vi "VIH HelpGen - Build.vi"(8 "error in":errorcluster, 9 "Allowed files":path[](array[path]), 10 "Items Array":T3[](array[typedef]), 11 "Project Tree":T2) -> (0 "error out":errorcluster, 2 "Items out":T1, 3 "dup Project Tree":T2)   [LabVIEW 2014]
doc: "::: VI Helpeks :::\nCopyright (c) 2000-2026 Konstantin Shifershteyn. All rights reserved."
uses:
  _VIH HelpGen - Palette.llb/VIH HelpGen Typedef - Palette - Item Info Cluster.ctl
  _VIH HelpGen - Palette.llb/VIH HelpGen Typedef - Palette - Item Type Enum.ctl
  _VIH Project Manager.llb/VIH Project Tree Typedef - Tree Refnum.ctl
panel:
  # "VI Helpeks\nCopyright (c) 2012-2026 Konstantin Shifershteyn"
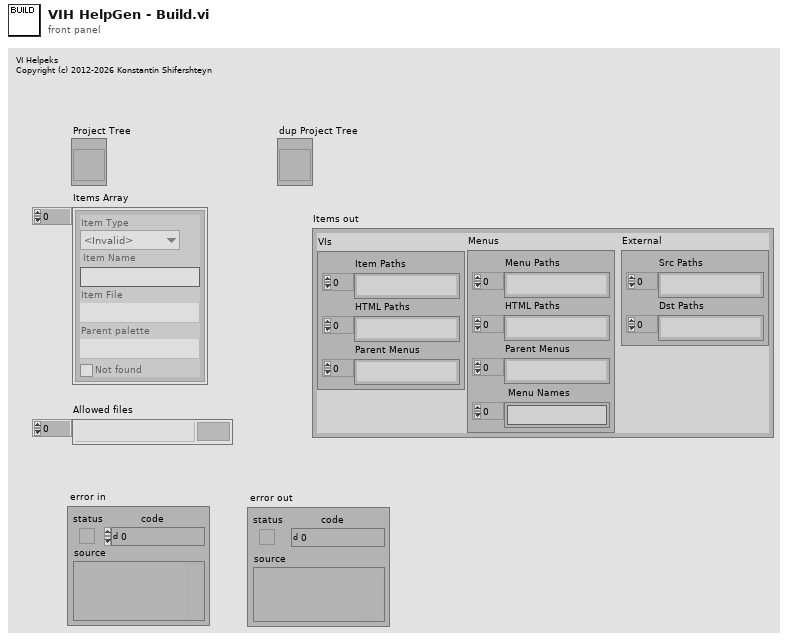
[diagram p1: front panel]
types:
  T1 = cluster{"VIs":cluster{"Item Paths":path[], "HTML Paths":path[], "Parent Menus":path[]}, "Menus":cluster{"Menu Paths":path[], "HTML Paths":path[], "Parent Menus":path[], " Menu Names":string[]}, "External":cluster{"Src Paths":path[], "Dst Paths":path[]}}
  T2 = typedef "VIH Project Tree Typedef - Tree Refnum.ctl" = refnum<vi>
  T3 = typedef "VIH HelpGen Typedef - Palette - Item Info Cluster.ctl" = cluster{"Item Type":T4, "Item Name":string, "Item File":path, "Parent palette":path, "Not found":bool}
  T4 = typedef "VIH HelpGen Typedef - Palette - Item Type Enum.ctl" = enum32{"<Invalid>", "<unknown>", "VI", "Menu", "LV Func", "Express VI", "Poly VI", "CTL", "HTML"}
  T5 = enum16{"nop", "Start", "Stop", "Run-prep", "Run-VI", "Run-Menu"}
  T6 = cluster{"Menu Paths":path[], "HTML Paths":path[], "Parent Menus":path[], " Menu Names":string[]}
  T7 = cluster{"Item Paths":path[], "HTML Paths":path[], "Parent Menus":path[]}
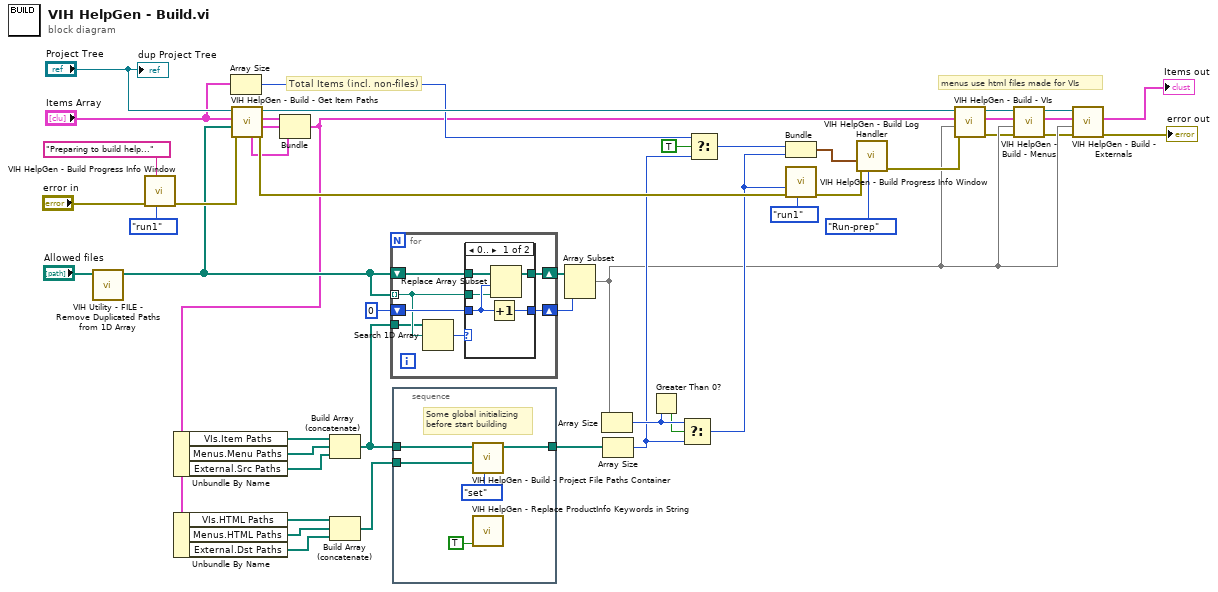
[diagram p0: block diagram]
diagram:
  # "menus use html files made for VIs"
  # "Total Items (incl. non-files)"
  n1 = call "VIH Utility - FILE - Remove Duplicated Paths from 1D Array.vi"("Array in"="Allowed files") -> ("Array out"=w25:path[])  [unwired: 9 in, 1 out]
  n2 = call "VIH HelpGen - Build Progress Info Window.vi"("Mode (run1)"=enum16{"start", "stop", "run1", "run2"}."run1" ("Mode (run)"), "Message"="Preparing to build help...", "error in"="error in") -> ("error out"=w45:errorcluster)  [unwired: 8 in]
  n3 = Array Size(array="Items Array") -> (size(s)=w23:i32)
  n4 = call "VIH HelpGen - Build - Get Item Paths.vi"("error in"=w45, "Allowed files"=w25, "Items Array"="Items Array", "Project Tree"="Project Tree") -> ("error out"=w26:errorcluster, "Menus"=w40:T6, "VIs"=w41:T7, "dup Project Tree"=w42:T2, "External"=w19:cluster{"Src Paths":path[], "Dst Paths":path[]})  [unwired: 3 in]
  n5 = Bundle("VIs"=w41, "Menus"=w40, "External"=w19) -> (w17:T1)  [unwired: 1 in]
  n6 = Unbundle By Name(w17) -> ("VIs.Item Paths"=w35:path[], "Menus.Menu Paths"=w34:path[], "External.Src Paths"=w18:path[])
  n7 = Unbundle By Name(w17) -> ("VIs.HTML Paths"=w16:path[], "Menus.HTML Paths"=w15:path[], "External.Dst Paths"=w14:path[])
  n8 = Build Array (concatenate)(w35, w34, w18) -> (w13:path[])
  n9 = Build Array (concatenate)(w16, w15, w14) -> (w12:path[])
  n10 = for {
    tunnel: w25 -> [w50] mode=indexing
    shift-right: [w53] -> w33
    shift-left: w25 -> [w54]
    shift-right: [w51] -> w32
    shift-left: 0 -> [w52]
    tunnel: w13 -> [w49]
    n11 = Search 1D Array(1D array=w49, element=w50) -> (index of element=w48:i32)  [unwired: 1 in]
    n12 = case shown="0.." w48 {
      tunnel: w54 -> [w59 w61]
      tunnel: [w56 w61] -> w53
      tunnel: w52 -> [w58 w60]
      tunnel: [w57 w60] -> w51
      tunnel: w50 -> [w55 _]
      frame 0.. {
        n13 = Increment(x=w58) -> (x+1=w57:i32)
        n14 = Replace Array Subset(array=w59, new element=w55, index=w58) -> (w56:path[])
      }
      frame ..-1 {
      }
    }
  }
  n15 = stacked-sequence {
    tunnel: w13 -> [w66]
    tunnel: w12 -> [w65]
    tunnel: [w63] -> w11
    frame #0 {
      # "Some global initializing\nbefore start building"
      n16 = call "VIH HelpGen - Build - Project File Paths Container.vi"("cmd (get)"=enum16{"get", "set"}."set", "HTML Paths in"=w65, "Item Paths in"=w66) -> ("Item Paths"=w63:path[])  [unwired: 6 in, 2 out]
      n17 = call "VIH HelpGen - Replace ProductInfo Keywords in String.vi"("Init (F)"=TRUE) -> ()  [unwired: 10 in, 1 out]
    }
  }
  n18 = Array Subset(array=w33, length=w32) -> (w9:path[])  [unwired: 1 in]
  n19 = Array Size(array=w9) -> (size(s)=w30:i32)
  n20 = Array Size(array=w11) -> (size(s)=w22:i32)
  n21 = Greater Than 0?(x=w30) -> (x > 0?=w29:bool)
  n22 = Select(t=w30, s=w29, f=w22) -> (s? t:f=w20:i32)
  n23 = Select(t=w23, s=TRUE, f=w22) -> (s? t:f=w21:i32)
  n24 = Bundle(w21, w20) -> (w7:cluster{i32, i32})  [unwired: 1 in]
  n25 = call "VIH HelpGen - Build Progress Info Window.vi"("Mode (run1)"=enum16{"start", "stop", "run1", "run2"}."run1" ("Mode (run)"), "error in"=w26, "# steps"=w20) -> ("error out"=w28:errorcluster)  [unwired: 8 in]
  n26 = call "VIH HelpGen - Build Log Handler.vi"("cmd (nop)"=T5."Run-prep" ("cmd"), "error in"=w28, "Files #"=w7) -> ("error out"=w27:errorcluster)  [unwired: 4 in, 4 out]
  n27 = call "VIH HelpGen - Build - VIs.vi"("error in"=w27, "File paths"=w9, "Items"=w17, "Project Tree"=w42) -> ("error out"=w4:errorcluster, "Items out"=w6:T1, "dup Project Tree"=w5:T2)  [unwired: 5 in]
  n28 = call "VIH HelpGen - Build - Menus.vi"("error in"=w4, "File paths"=w9, "Items"=w6, "Project Tree"=w5) -> ("error out"=w3:errorcluster, "Items out"=w1:T1, "dup Project Tree"=w2:T2)  [unwired: 5 in]
  n29 = call "VIH HelpGen - Build - Externals.vi"("error in"=w3, "File paths"=w9, "Items"=w1, "Project Tree"=w2) -> ("error out"=→"error out":errorcluster, "Items out"=→"Items out":T1)  [unwired: 5 in, 1 out]
  "dup Project Tree" <- "Project Tree"
